vi "揭晓游戏结局.vi"(1 "地图":i32[][](array[numeric])) -> (0 "输出地图":i32[][](array[numeric]))   [LabVIEW 2017]
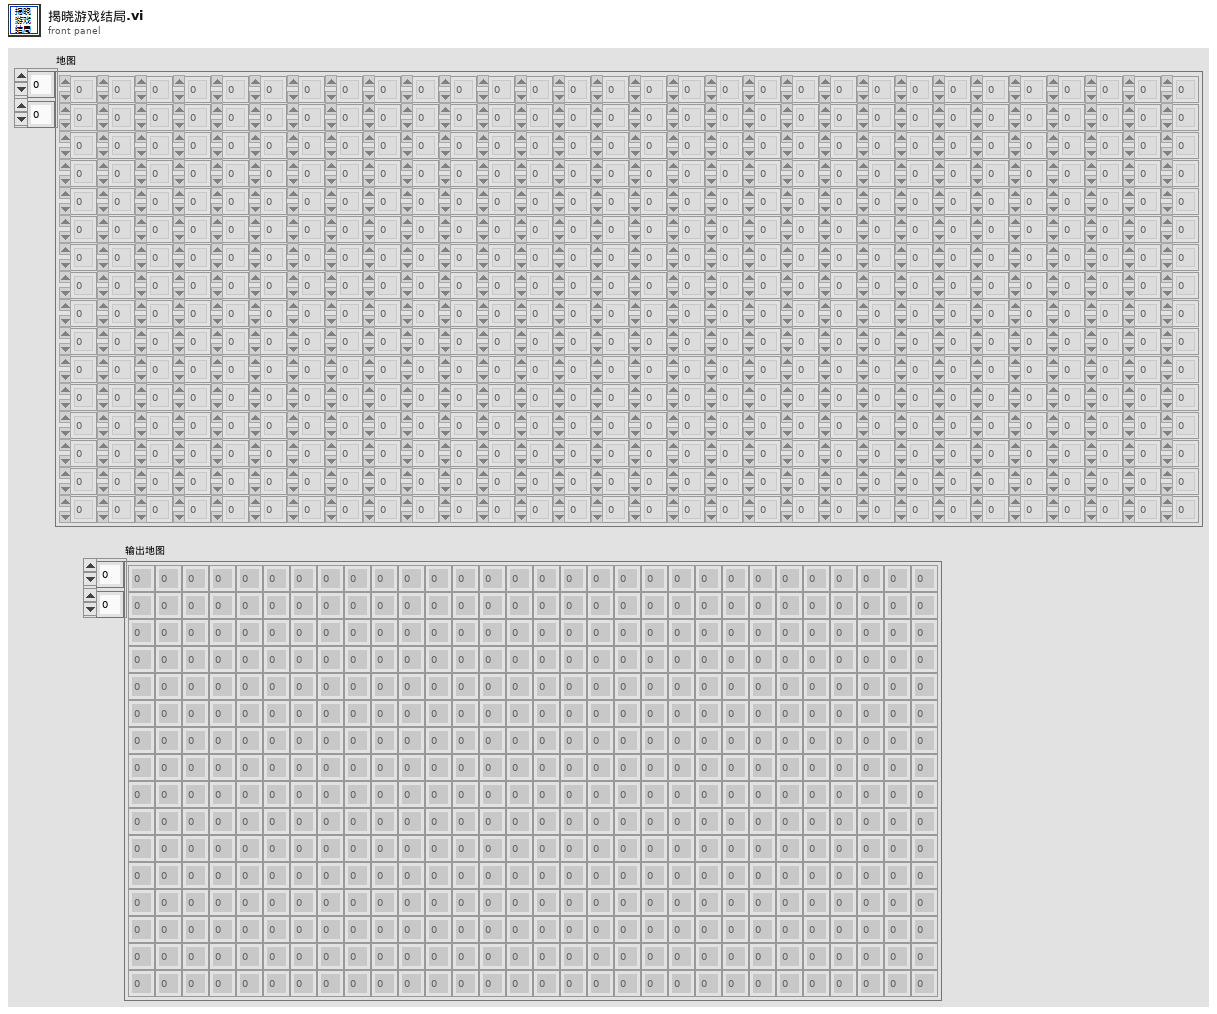
[diagram p1: front panel]
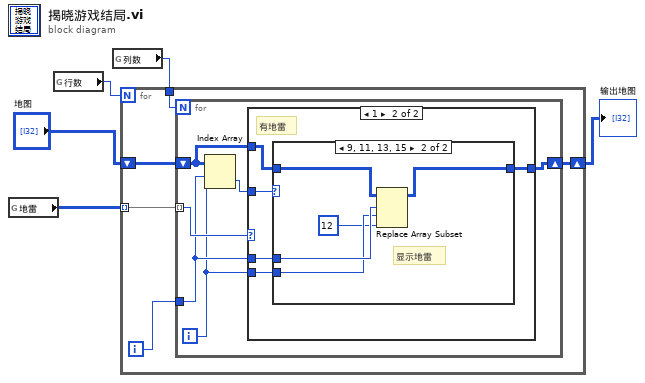
[diagram p0: block diagram]
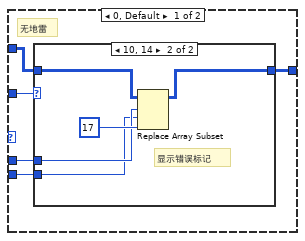
[diagram p2: hidden frame]
diagram:
  n1 = global read "全局变量.vi" "地雷"() -> (w3:i16[][])
  n2 = global read "全局变量.vi" "行数"() -> (w2:i32)
  n3 = global read "全局变量.vi" "列数"() -> (w1:i32)
  n4 = for {
    N: w2 -> [_]
    shift-right: [w9] -> w5
    shift-left: "地图" -> [w10]
    tunnel: w3 -> [w7] mode=indexing
    tunnel: w1 -> [w6]
    i -> [w8]
    n5 = for {
      N: w6 -> [_]
      shift-right: [w13] -> w9
      shift-left: w10 -> [w14]
      tunnel: w8 -> [w12]
      tunnel: w7 -> [w15] mode=indexing
      i -> [w11]
      n6 = Index Array(array=w14, index (row)=w12, index (col)=w11) -> (element=w16:i32)
      n7 = case shown="1" w15 {
        tunnel: w16 -> [w19 w32]
        tunnel: w14 -> [w20 w31]
        tunnel: [w21 w30] -> w13
        tunnel: w12 -> [w18 w29]
        tunnel: w11 -> [w17 w28]
        frame 0, Default {
          # "无地雷"
          n8 = case shown="10, 14" w19 {
            tunnel: [w22 w24] -> w21
            tunnel: w20 -> [w22 w23]
            tunnel: w18 -> [_ w26]
            tunnel: w17 -> [_ w25]
            frame 0, Default {
            }
            frame 10, 14 {
              # "显示错误标记"
              n9 = Replace Array Subset(array=w23, new element=17, index (row)=w26, index (col)=w25) -> (w24:i32[][])
            }
          }
        }
        frame 1 {
          # "有地雷"
          n10 = case shown="9, 11, 13, 15" w32 {
            tunnel: w31 -> [w33 w38]
            tunnel: [w33 w37] -> w30
            tunnel: w29 -> [_ w36]
            tunnel: w28 -> [_ w35]
            frame 0..8, Default {
              # "无地雷，不可能的情况"
            }
            frame 9, 11, 13, 15 {
              # "显示地雷"
              n11 = Replace Array Subset(array=w38, new element=12, index (row)=w36, index (col)=w35) -> (w37:i32[][])
            }
          }
        }
      }
    }
  }
  "输出地图" <- w5
